vi "Get Message Placement Cluster.vi"(6 "Is Serialization Cluster":bool=TRUE, 7 "MessageElementMetadata":T1, 8 "error in (no error)":errorcluster, 10 "VI in":refnum<vi>, 11 "Library":refnum<vi>) -> (0 "error out":errorcluster, 1 "Control ref out":refnum<vi>, 2 "VI out":refnum<vi>, 3 "Library item out":refnum<vi>, 5 "LVClassLibrary Refnum":refnum<vi>)   [LabVIEW 2019, in "gRPC Template Creation Utility.lvlib"]
uses:
  gRPC Template Creation Utility.lvlib
  TypeDefs/Message Element Metadata (Scripting).ctl
  TypeDefs/Message Element Type.ctl
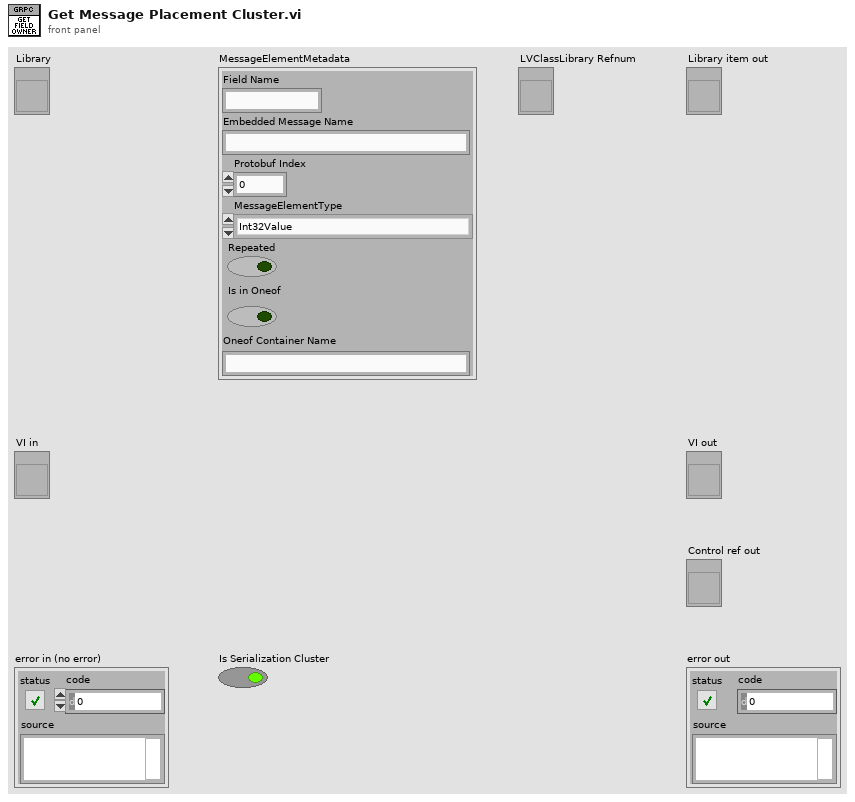
[diagram p1: front panel]
types:
  T1 = typedef "gRPC Template Creation Utility.lvlib/Message Element Metadata (Scripting).ctl" = cluster{"Field Name":string, "Embedded Message Name":string, "Protobuf Index":i32, "MessageElementType":T2, "Repeated":bool, "Is in Oneof":bool, "Oneof Container Name":string}
  T2 = typedef "gRPC Template Creation Utility.lvlib/Message Element Type.ctl" = enum32{"Int32Value", "FloatValue", "DoubleValue", "BoolValue", "StringValue", "MessageValue", "Int64Value", "UInt32Value", "UInt64Value", "EnumValue", "Bytes", "Fixed64", "Fixed32", "SFixed64", "SFixed32", "SInt64", "SInt32"}
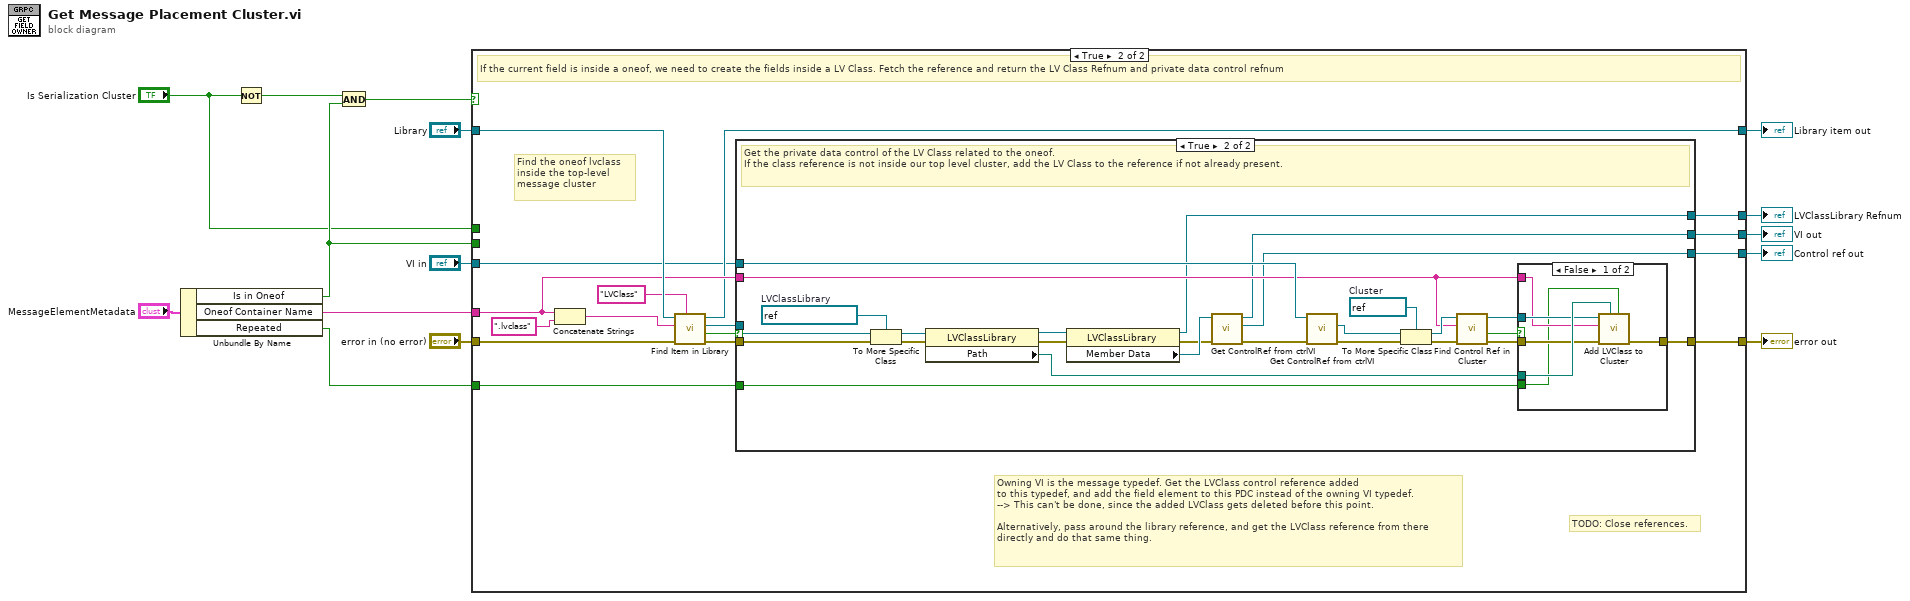
[diagram p0: block diagram]
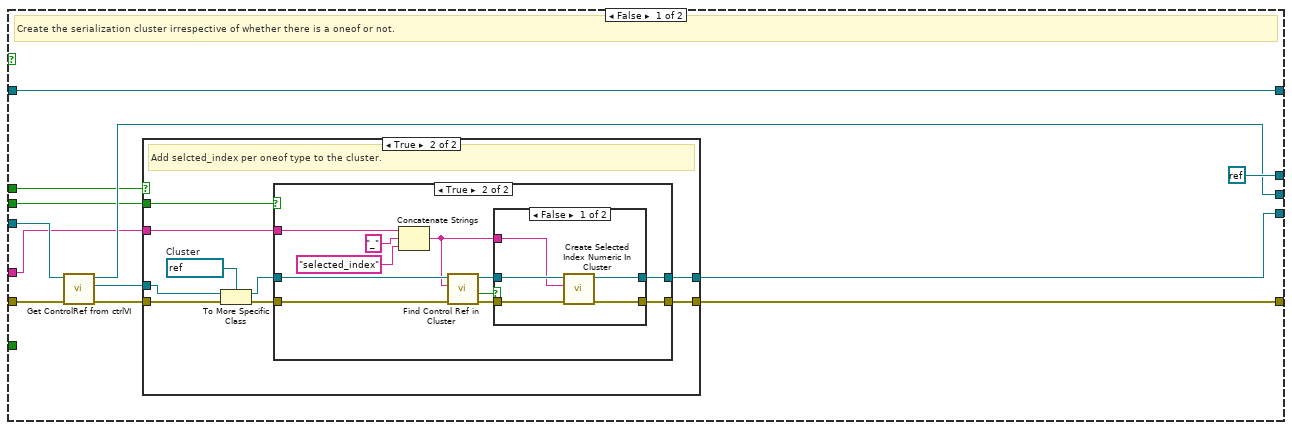
[diagram p2: hidden frame]
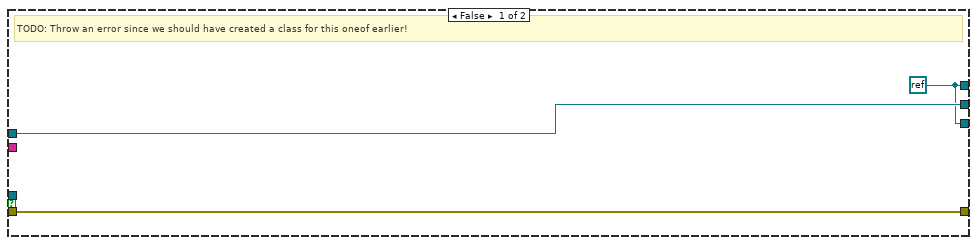
[diagram p6: hidden frame]
diagram:
  n1 = Unbundle By Name("MessageElementMetadata") -> ("Is in Oneof"=w3:bool, "Oneof Container Name"=w8:string, "Repeated"=w1:bool)
  n2 = Not(x="Is Serialization Cluster") -> (.not. x?=w4:bool)
  n3 = And(x=w4, y=w3) -> (x .and. y?=w6:bool)
  n4 = case shown="True" w6 {
    tunnel: w8 -> [w20 w67]
    tunnel: "VI in" -> [w25 w61]
    tunnel: "error in (no error)" -> [w23 w73]
    tunnel: [w24 w65] -> w13
    tunnel: [w18 w64] -> w15
    tunnel: "Library" -> [w27 w74]
    tunnel: [w27 w63] -> w12
    tunnel: [w21 w62] -> w14
    tunnel: [refnum<k0> refnum w60] -> w5
    tunnel: w3 -> [w17 _]
    tunnel: "Is Serialization Cluster" -> [w16 _]
    tunnel: w1 -> [_ w59]
    frame False {
      # "Create the serialization cluster irrespective of whether there is a oneof or not."
      n5 = call "Get ControlRef from ctrlVI.vi"("error in (no error)"=w23, "VI ref in"=w25) -> ("error out"=w19:errorcluster, "Control ref out"=w22:refnum<vi>, "VI ref out"=w24:refnum<vi>)  [unwired: 7 in]
      n6 = case shown="True" w16 {
        tunnel: w22 -> [w29 w38]
        tunnel: [w29 w34] -> w21
        tunnel: w20 -> [_ w35]
        tunnel: w19 -> [w28 w33]
        tunnel: [w28 w31] -> w18
        tunnel: w17 -> [_ w30]
        frame False {
        }
        frame True {
          w37 = refnum<vi> refnum  # Cluster
          # "Add selcted_index per oneof type to the cluster."
          n7 = To More Specific Class(target class=w37, reference=w38, error in=w33) -> (specific class reference=w36:refnum<vi>, error out=w32:errorcluster)
          n8 = case shown="True" w30 {
            tunnel: w36 -> [w39 w51]
            tunnel: w35 -> [_ w48]
            tunnel: [w39 w44] -> w34
            tunnel: w32 -> [w40 w42]
            tunnel: [w40 w41] -> w31
            frame False {
            }
            frame True {
              n9 = Concatenate Strings(w48, "_" ("string"), "selected_index" ("Control Name")) -> (w43:string)
              n10 = call "Find Control Ref in Cluster.vi"("error in (no error)"=w42, "Control Name"=w43, "Cluster ref in"=w51) -> ("error out"=w46:errorcluster, "Found ?"=w47:bool, "Cluster ref out"=w45:refnum<vi>)  [unwired: 5 in, 1 out]
              n11 = case shown="False" w47 {
                tunnel: w46 -> [w56 w58]
                tunnel: [w53 w58] -> w41
                tunnel: w45 -> [w55 w57]
                tunnel: [w54 w57] -> w44
                tunnel: w43 -> [w52 _]
                frame False {
                  n12 = call "Create Selected Index Numeric In Cluster.vi"("error in (no error)"=w56, "Label.Text"=w52, "Cluster in"=w55) -> ("error out"=w53:errorcluster, "Cluster out"=w54:refnum<vi>)  [unwired: 7 in]
                }
                frame True {
                }
              }
            }
          }
        }
      }
    }
    frame True {
      # "Find the oneof lvclass \ninside the top-level \nmessage cluster"
      # "TODO: Close references."
      # "Owning VI is the message typedef. Get the LVClass control reference added\nto this typedef, and add the field element to this PDC instead of the owning VI typedef.\n--> This can't be done, since the added LVClass gets deleted before this point.\n\nAlternatively, pass around the library reference, and get the LVClass reference from there\ndirectly and do that same thing."
      # "If the current field is inside a oneof, we need to create the fields inside a LV Class. Fetch the reference and return the LV Class Refnum and private data control refnum"
      n13 = Concatenate Strings(w67, ".lvclass" ("string")) -> (w72:string)
      n14 = call "Find Item in Library.vi"("Item Type"="LVClass", "error in (no error)"=w73, "Item Name"=w72, "Library item in"=w74) -> ("error out"=w68:errorcluster, "Found?"=w70:bool, "Project Item (Library Item)"=w69:refnum<vi>, "Library item out"=w63:refnum<vi>)  [unwired: 4 in]
      n15 = case shown="True" w70 {
        tunnel: w69 -> [_ w97]
        tunnel: w68 -> [w76 w98]
        tunnel: w61 -> [w77 w102]
        tunnel: w67 -> [_ w89]
        tunnel: [w77 w83] -> w65
        tunnel: [w76 w84] -> w64
        tunnel: [w75 w82] -> w62
        tunnel: [w75 w88] -> w60
        tunnel: w59 -> [_ w78]
        frame False {
          w75 = refnum<k0> refnum
          # "TODO: Throw an error since we should have created a class for this oneof earlier!"
        }
        frame True {
          w96 = refnum<vi> refnum  # LVClassLibrary
          w100 = refnum<vi> refnum  # Cluster
          # "Get the private data control of the LV Class related to the oneof. \nIf the class reference is not inside our top level cluster, add the LV Class to the reference if not already present."
          n16 = To More Specific Class(target class=w96, reference=w97, error in=w98) -> (specific class reference=w95:refnum<vi>, error out=w94:errorcluster)
          n17 = property class="LVClassLibrary"(reference=w95, error in=w94) -> (reference out=w93:refnum<vi>, error out=w92:errorcluster, "Path"=w103:path)
          n18 = property class="LVClassLibrary"(reference=w93, error in=w92) -> (reference out=w88:refnum<vi>, error out=w86:errorcluster, "Member Data"=w87:refnum<vi>)
          n19 = call "Get ControlRef from ctrlVI.vi"("error in (no error)"=w86, "VI ref in"=w87) -> ("error out"=w85:errorcluster, "Control ref out"=w82:refnum<vi>, "VI ref out"=w83:refnum<vi>)  [unwired: 7 in]
          n20 = call "Get ControlRef from ctrlVI.vi"("error in (no error)"=w85, "VI ref in"=w102) -> ("error out"=w99:errorcluster, "Control ref out"=w101:refnum<vi>)  [unwired: 7 in, 1 out]
          n21 = To More Specific Class(target class=w100, reference=w101, error in=w99) -> (specific class reference=w90:refnum<vi>, error out=w91:errorcluster)
          n22 = call "Find Control Ref in Cluster.vi"("error in (no error)"=w91, "Control Name"=w89, "Cluster ref in"=w90) -> ("error out"=w80:errorcluster, "Found ?"=w79:bool, "Cluster ref out"=w81:refnum<vi>)  [unwired: 5 in, 1 out]
          n23 = case shown="False" w79 {
            tunnel: w103 -> [w109 _]
            tunnel: [w108 w110] -> w84
            tunnel: w81 -> [w107 _]
            tunnel: w89 -> [w106 _]
            tunnel: w80 -> [w105 w110]
            tunnel: w78 -> [w104 _]
            frame False {
              n24 = call "Add LVClass to Cluster.vi"("isArray (F)"=w104, "LVClass path"=w109, "error in (no error)"=w105, "Field Name"=w106, "Owning cluster ref in"=w107) -> ("error out"=w108:errorcluster)  [unwired: 4 in, 2 out]
            }
            frame True {
            }
          }
        }
      }
    }
  }
  "LVClassLibrary Refnum" <- w5
  "error out" <- w15
  "Control ref out" <- w14
  "VI out" <- w13
  "Library item out" <- w12
